vi "1m forward.vi"   [LabVIEW 2017]
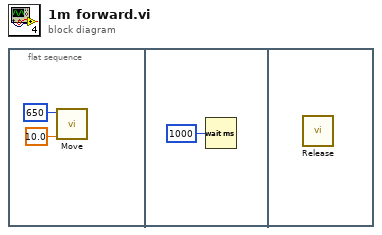
[diagram p0: block diagram]
diagram:
  n1 = flat-sequence {
    frame #0 {
      n2 = call "Move.vi"("Speed (0-30)"=10.0, "Distance (mm)"=650) -> ()  [unwired: 8 in]
    }
    frame #1 {
      n3 = Wait (ms)(milliseconds to wait=u32 1000) -> ()  [unwired: 1 out]
    }
    frame #2 {
      n4 = call "Release.vi"() -> ()  [unwired: 12 in]
    }
  }
